vi "get channel info.vi"(1 "device type":T2=enum."LAN") -> (0 "channel info":T1={"number of physical channels"=1, "peakcan channel base code"=0} {"peakcan channel base code" format="%x"})   [LabVIEW 2024]
doc: "Gets channel information for a specific device type."
uses:
  device type.ctl
  channel info.ctl
  atsj peakcan basic.lvlib
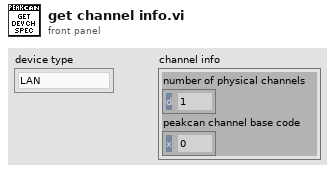
[diagram p1: front panel]
types:
  T1 = typedef "channel info.ctl" = cluster{"number of physical channels":u8, "peakcan channel base code":u16}
  T2 = typedef "atsj peakcan basic.lvlib/device type.ctl" = enum8{"ISA", "DNG", "PCI", "USB", "PCC", "LAN"}
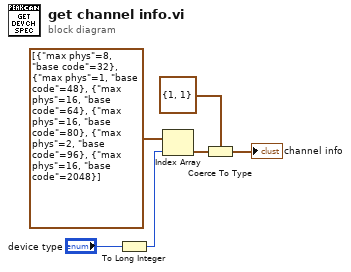
[diagram p0: block diagram]
diagram:
  n1 = To Long Integer(number="device type") -> (32bit integer=w4:i32)
  n2 = Index Array(array=cluster{"max phys":u8, "base code":u16}[] [{"max phys"=8, "base code"=32}, {"max phys"=1, "base code"=48}, {"max phys"=16, "base code"=64}, {"max phys"=16, "base code"=80}, {"max phys"=2, "base code"=96}, {"max phys"=16, "base code"=2048}], index=w4) -> (element=w3:cluster{"max phys":u8, "base code":u16})
  n3 = Coerce To Type(0:w3, 1:T1 {"number of physical channels"=1, "peakcan channel base code"=1}) -> (2:→"channel info":T1)
